vi "Sample.vi"(8 "错误输入（无错误）":errorcluster, 10 "基本信息":T1={"USB Port"="", "采集间隔(s)"=0.5, "位置"=0, "速度(r/min)"=70}) -> (0 "错误输出":errorcluster, 2 "PoNSp":dbl[](array[numeric]))   [LabVIEW 2026, in "UI-步进.lvlib" / "Acquisition.lvlib"]
uses:
  Acquisition.lvlib
  Supports/Sample Settings.ctl
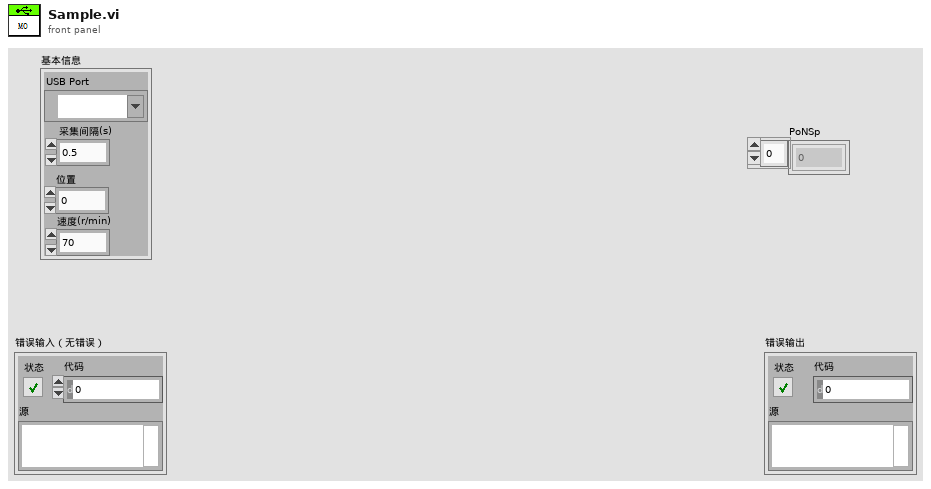
[diagram p1: front panel]
types:
  T1 = typedef "UI-步进.lvlib/Sample Settings.ctl" = cluster{"USB Port":refnum<visa-resource-name>, "采集间隔(s)":dbl, "位置":i32, "速度(r/min)":i32}
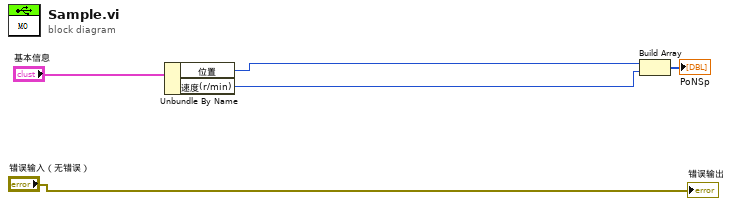
[diagram p0: block diagram]
diagram:
  n1 = Unbundle By Name("基本信息") -> ("位置"=w2:i32, "速度(r/min)"=w1:i32)
  n2 = Build Array(w2, w1) -> (→"PoNSp":i32[])
  "错误输出" <- "错误输入（无错误）"
